vi "Draw Markers.vi"(8 "error in (no error)":errorcluster, 11 "SequenceViewPanel in":refnum<class "SequenceViewPanel.lvclass">) -> (0 "error out":errorcluster, 2 "Markers":picture, 3 "SequenceViewPanel out":refnum<class "SequenceViewPanel.lvclass">)   [LabVIEW 2020, in "TSnax UI.lvlib" / "SequenceViewPanel.lvclass"]
uses:
  SequenceViewPanel.lvclass
  SequenceViewPanel.lvclass/SequenceViewPanel.ctl
  Image.ctl
  TSnax UI Manager/TSnax UI Manager.lvclass
  TSnax UI.lvlib
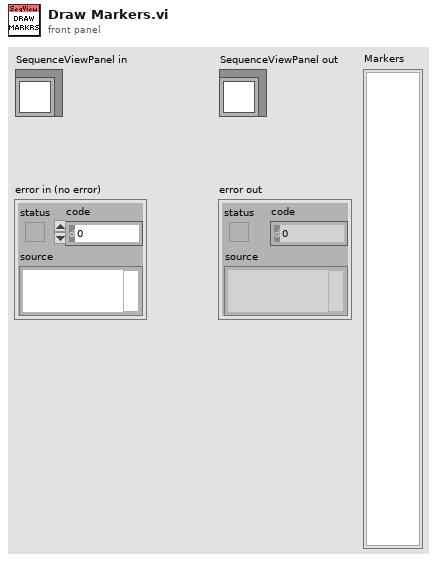
[diagram p1: front panel]
types:
  T1 = typedef "TSnax UI.lvlib/SequenceViewPanel.lvclass/Ref Data.ctl" = cluster{"Insert Line":i32, "SequenceFile":refnum<class "SequenceFile.lvclass">, "Sequence":string, "Trace Marker":i32}
  T2 = typedef "TSnax UI.lvlib/Image.ctl" = enum16{"YellowArrow", "GreenArrow"}
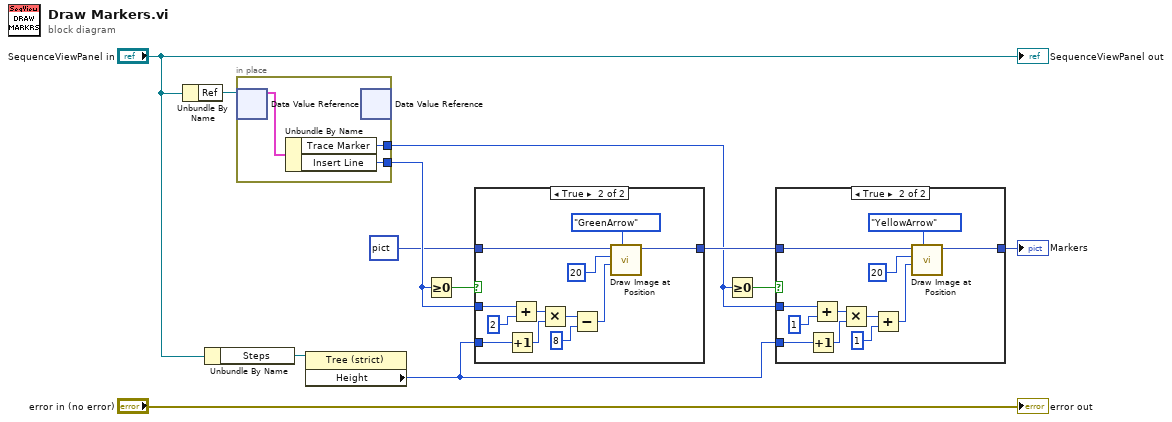
[diagram p0: block diagram]
diagram:
  n1 = Unbundle By Name("SequenceViewPanel in") -> ("Ref"=w10:refnum<data-value>)
  n2 = Unbundle By Name("SequenceViewPanel in") -> ("Steps"=w11:refnum<vi>)
  n3 = in-place {
    in-place-border: [w14] -> w8
    in-place-border: [w13] -> w3
    n4 = in-place-dvr #1(w10) -> (w15:T1)  [unwired: 1 out]
    n5 = Unbundle By Name(w15) -> ("Trace Marker"=w13:i32, "Insert Line"=w14:i32)
    n6 = in-place-dvr #1() -> ()  [unwired: 1 in, 2 out]
  }
  n7 = property class="Tree (strict)"(reference=w11) -> ("Height"=w2:i32)  [unwired: 1 in, 2 out]
  n8 = Greater Or Equal To 0?(x=w8) -> (x >= 0?=w7:bool)
  n9 = case shown="True" w7 {
    tunnel: w2 -> [_ w21]
    tunnel: [w16 w20] -> w4
    tunnel: w8 -> [_ w19]
    tunnel: picture data[5B] ("Picture") -> [w16 w18]
    frame False {
    }
    frame True {
      n10 = Increment(x=w21) -> (x+1=w17:i32)
      n11 = Add(x=w19, y=2) -> (x+y=w26:i32)
      n12 = Multiply(x=w26, y=w17) -> (x*y=w24:i32)
      n13 = Subtract(x=w24, y=8) -> (x-y=w22:i32)
      n14 = call "Draw Image at Position.vi"("Image"=Image."GreenArrow", "Top"=w22, "Left"=i16 20, "Picture In"=w18) -> ("Picture"=w20:picture)  [unwired: 7 in]
    }
  }
  n15 = Greater Or Equal To 0?(x=w3) -> (x >= 0?=w5:bool)
  n16 = case shown="True" w5 {
    tunnel: w2 -> [_ w34]
    tunnel: [w29 w33] -> w1
    tunnel: w3 -> [_ w32]
    tunnel: w4 -> [w29 w31]
    frame False {
    }
    frame True {
      n17 = Increment(x=w34) -> (x+1=w30:i32)
      n18 = Add(x=w32, y=1) -> (x+y=w39:i32)
      n19 = Multiply(x=w39, y=w30) -> (x*y=w37:i32)
      n20 = Add(x=w37, y=1) -> (x+y=w35:i32)
      n21 = call "Draw Image at Position.vi"("Image"=Image."YellowArrow", "Top"=w35, "Left"=i16 20, "Picture In"=w31) -> ("Picture"=w33:picture)  [unwired: 7 in]
    }
  }
  "Markers" <- w1
  "error out" <- "error in (no error)"
  "SequenceViewPanel out" <- "SequenceViewPanel in"
